vi "Scratch.vi"() -> ()   [LabVIEW 2020, in "VolatusSeq.lvlib"]
uses:
  VolatusSeq.lvlib
  Sequencing Status JSON.ctl
  Sequence Status JSON.ctl
  lv-web-crypto/lv-crypto/Crypto/Hashes/SHA-256/SHA-256.lvclass
  <vilib>/httpClient/MultipartData.ctl
  839e7588-aafe-4656-a2fc-0ebd197a9b7a.vi
  9333b484-011f-4693-912f-1257e8b2ee91.vi
  d0b18555-7aa2-4285-8466-e3de5a6bf30b.vi
  80ab21ca-ea82-40af-a504-7941cea15b69.vi
  <vilib>/JDP Science/JSONtext/Next JSON Value.vi
  <vilib>/JDP Science/JSONtext/String Subset.vi
  <vilib>/JDP Science/JSONtext/Parsing/Advance past next JSON Value (inlined COPY).vi
  <vilib>/JDP Science/JSONtext/Parsing/Advance past whitespace.vi
  <vilib>/JDP Science/JSONtext/Parsing/Advance past String.vi
  <vilib>/JDP Science/JSONtext/Parsing/Advance past Number.vi
  <vilib>/JDP Science/JSONtext/Parsing/Advance past Line Ending.vi
  <vilib>/JDP Science/JSONtext/Parsing/Parse Full Path or Item Name.vi
  <vilib>/JDP Science/JSONtext/Parsing/Advance past Array.vi
  <vilib>/JDP Science/JSONtext/Parsing/Advance past Object.vi
  <vilib>/JDP Science/JSONtext/support/Error Cluster From Code.vi
  <vilib>/JDP Science/JSONtext/Offset/Find Item Locations by Path.vi
  <vilib>/JDP Science/JSONtext/JSON text to Variant.vi
  <vilib>/JDP Science/JSONtext/LVClass Serializer/JSONtext LVClass Serializer.lvclass
  <vilib>/JDP Science/JSONtext/JSONtext.lvlib
  lv-web-crypto/lv-crypto/Crypto/Crypto.lvlib
  <vilib>/httpClient/LabVIEWHTTPClient.lvlib
  lv-vecto/Vecto/Vecto.lvlib
  lv-web-crypto/lv-json/JSON/JSON.lvlib
  ad4a9e69-8c40-4036-95cd-164e8a1331be.vi
panel:
  in  "URL Base":string="http://localhost:13083"
  out "Table":string[][](table)
  in  "Abort":bool
  in  "Unload":bool
  in  "Start":bool
  in  "Load":bool
  in  "VSEQ":string="{\n    \"Sequence\": {\n        \"Name\": \"Bottle Condition\",\n        \"Version\": \"1\",\n        \"Comment\": \"Control state machine for bottle heating/cooling.\",\n        \"Entry\": \"Start\",\n        \"Abort\": \"Stop\",\n        \"States\": {\n            \"Start\": {\n                \"Comment\": \"Reset bottle controls to off state.\",\n                \"Steps\": [\n                    {\n                        \"Time\": 0,\n                        \"Commands\": [\n                            {\"Type\": \"Transition\", \"Target\": \"Hold\"}\n                        ]\n                    }\n                ]\n            },\n            \"Hold\": {\n                \"Comment\": \"Bottle in range, controls off.\",\n                \"Steps\": [\n                    {\n                        \"Time\": 0,\n                        \"Commands\": [\n                            {\"Type\": \"Digital\", \"Channel\": \"BottleCool\", \"Value\": false},\n                            {\"Type\": \"Digital\", \"Channel\": \"BottleHeat\", \"Value\": false}\n                        ]\n                    }\n                ],\n                \"Transitions\": [\n                    {\n                        \"Type\": \"State\",\n                        \"Target\": \"Cool\",\n                        \"Logic\": \"Any\",\n                        \"Conditions\": [\n                            {\"Type\": \"HighLimit\", \"Channel\": \"BottlePSI\", \"Limit\": 850}\n                        ]\n                    },\n                    {\n                        \"Type\": \"State\",\n                        \"Target\": \"Heat\",\n                        \"Logic\": \"Any\",\n                        \"Conditions\": [\n                            {\"Type\": \"LowLimit\", \"Channel\": \"BottlePSI\", \"Limit\": 750}\n                        ]\n                    }\n                ]\n            },\n            \"Cool\": {\n                \"Comment\": \"Cooling, wait for pressure to drop.\",\n                \"Steps\": [\n                    {\n                        \"Time\": 0,\n                        \"Commands\": [\n                            {\"Type\": \"Digital\", \"Channel\": \"BottleCool\", \"Value\": true}\n                        ]\n                    }\n                ],\n                \"Transitions\": [\n                    {\n                        \"Type\": \"State\",\n                        \"Target\": \"Start\",\n                        \"Logic\": \"Any\",\n                        \"Conditions\": [\n                            {\"Type\": \"LowLimit\", \"Channel\": \"BottlePSI\", \"Limit\": 800}\n                        ]\n                    }\n                ]\n            },\n            \"Heat\": {\n                \"Comment\": \"Heating, wait for pressure to rise.\",\n                \"Steps\": [\n                    {\n                        \"Time\": 0,\n                        \"Commands\": [\n                            {\"Type\": \"Digital\", \"Channel\": \"BottleHeat\", \"Value\": true}\n                        ]\n                    }\n                ],\n                \"Transitions\": [\n                    {\n                        \"Type\": \"State\",\n                        \"Target\": \"Start\",\n                        \"Logic\": \"Any\",\n                        \"Conditions\": [\n                            {\"Type\": \"HighLimit\", \"Channel\": \"BottlePSI\", \"Limit\": 800}\n                        ]\n                    }\n                ]\n            },\n            \"Stop\": {\n                \"Comment\": \"Stopping, ensure controls off.\",\n                \"Steps\": [\n                    {\n                        \"Time\": 0,\n                        \"Commands\": [\n                            {\"Type\": \"Digital\", \"Channel\": \"BottleCool\", \"Value\": false},\n                            {\"Type\": \"Digital\", \"Channel\": \"BottleHeat\", \"Value\": false},\n                            {\"Type\": \"Stop\"}\n                        ]\n                    }\n                ]\n            }\n        }\n    }\n}"
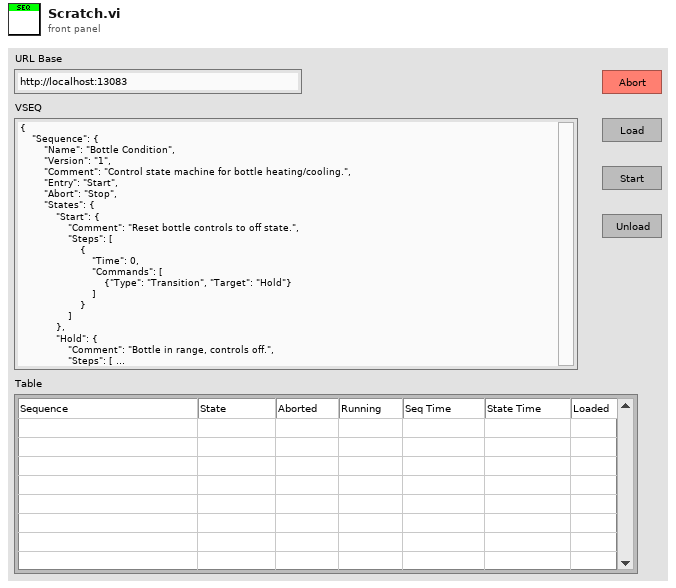
[diagram p1: front panel]
types:
  T1 = typedef "VolatusSeq.lvlib/Sequencing Status JSON.ctl" = cluster{"sequences":T2[]}
  T2 = typedef "VolatusSeq.lvlib/Sequence Status JSON.ctl" = cluster{"name":string, "state":string, "running":bool, "abort":bool, "time":cluster{"seq":i64, "state":i64, "wall":i64}, "loaded":bool, "started":i64, "crc":u32, "color_bg":string, "color_fg":string}
  T3 = typedef "LabVIEWHTTPClient.lvlib/MultipartData.ctl" = cluster{"Name":string, "Value":string, "File":path, "Filename":string, "MIME type":string}
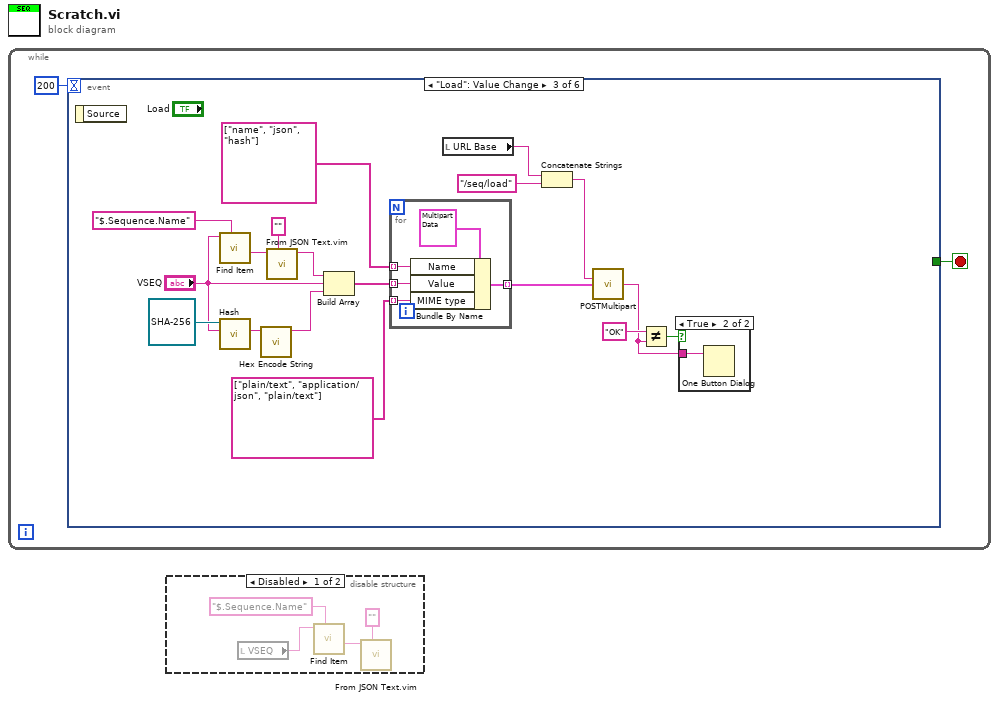
[diagram p0: block diagram]
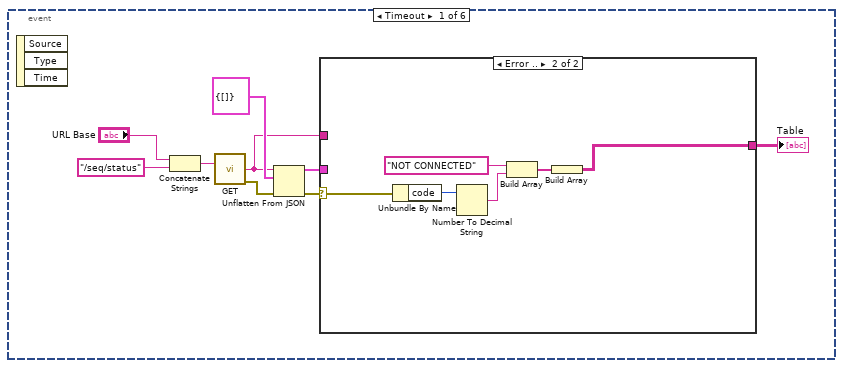
[diagram p3: hidden frame]
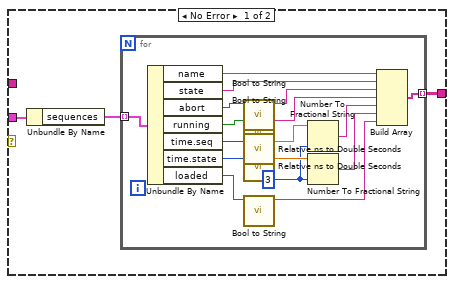
[diagram p4: hidden frame]
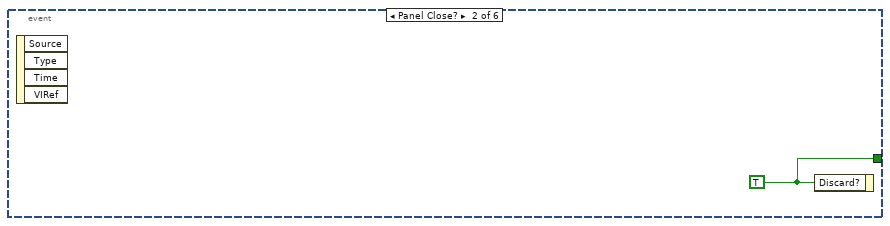
[diagram p5: hidden frame]
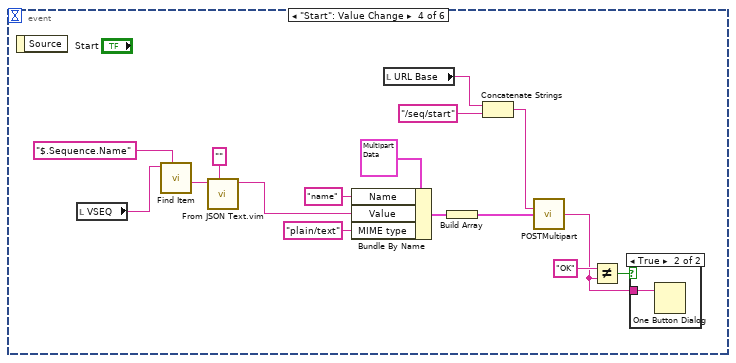
[diagram p7: hidden frame]
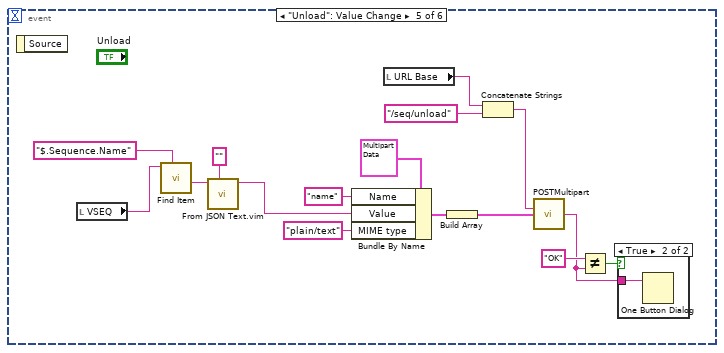
[diagram p9: hidden frame]
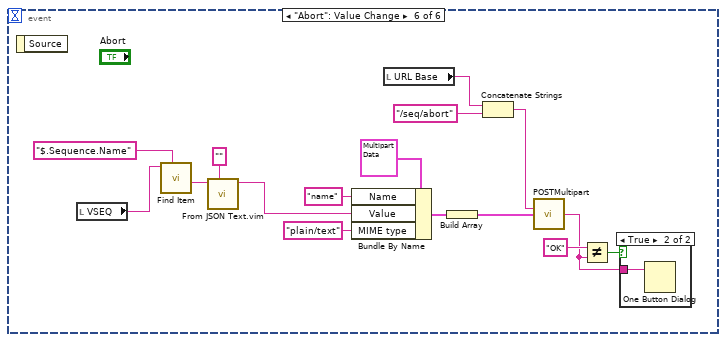
[diagram p11: hidden frame]
diagram:
  n1 = while {
    stop <- w1 stop-if-true
    n2 = event shown="[2] \"Load\": Value Change" {
      selector: _ -> [_ _ _ _ _ _]
      dyn-events: _ -> [_ _ _ _ _ _]
      timeout: 200 -> [_ _ _ _ _ _]
      tunnel: [_ w38 _ _ _ _] -> w1
      event Timeout {
        n3 = event-data() -> ()  [unwired: 1 in, 3 out]
        n4 = Concatenate Strings("URL Base", "/seq/status" ("string")) -> (w9:string)
        n5 = call <vilib>:"GET.vi"("url"=w9) -> ("body"=w3:string, "error out"=w8:errorcluster)  [unwired: 11 in, 2 out]
        n6 = Unflatten From JSON(JSON string=w3, type and defaults=T1 {"sequences"=[]} ("Sequencing Status JSON"), error in (no error)=w8) -> (value=w6:T1, error out=w4:errorcluster)  [unwired: 4 in]
        n7 = case shown="Error .." w4 {
          selector: w4 -> [_ w37]
          tunnel: w6 -> [w14 _]
          tunnel: [w12 w32] -> w5
          tunnel: w3 -> [_ _]
          frame No Error {
            n8 = Unbundle By Name(w14) -> ("sequences"=w13:T2[])
            n9 = for {
              tunnel: w13 -> [w31] mode=indexing
              tunnel: [w17] -> w12 mode=indexing
              w25 = i16 3 ("precision (6)")
              n10 = Unbundle By Name(w31) -> ("name"=w23:string, "state"=w22:string, "abort"=w28:bool, "running"=w27:bool, "time.seq"=w30:i64, "time.state"=w29:i64, "loaded"=w16:bool)
              n11 = call "Bool to String.vi"("Boolean"=w28) -> ("Value"=w21:string)  [unwired: 10 in]
              n12 = call "Bool to String.vi"("Boolean"=w27) -> ("Value"=w20:string)  [unwired: 10 in]
              n13 = call "Relative ns to Double Seconds.vi"("relative ns"=w30) -> ("Double s"=w24:dbl)  [unwired: 6 in]
              n14 = call "Relative ns to Double Seconds.vi"("relative ns"=w29) -> ("Double s"=w26:dbl)  [unwired: 6 in]
              n15 = call "Bool to String.vi"("Boolean"=w16) -> ("Value"=w15:string)  [unwired: 10 in]
              n16 = Number To Fractional String(number=w24, precision (6)=w25) -> (F-format string=w19:string)  [unwired: 2 in]
              n17 = Number To Fractional String(number=w26, precision (6)=w25) -> (F-format string=w18:string)  [unwired: 2 in]
              n18 = Build Array(w23, w22, w21, w20, w19, w18, w15) -> (w17:string[])
            }
          }
          frame Error {
            n19 = Unbundle By Name(w37) -> ("code"=w36:i32)
            n20 = Number To Decimal String(number=w36) -> (decimal integer string=w34:string)  [unwired: 1 in]
            n21 = Build Array("NOT CONNECTED", w34) -> (w33:string[])
            n22 = Build Array(w33) -> (w32:string[][])
          }
        }
        "Table" <- w5
      }
      event Panel Close? {
        w38 = TRUE ("Discard?")
        n23 = event-data() -> ()  [unwired: 1 in, 4 out]
        n24 = event-data("Discard?"=w38) -> ()  [unwired: 1 in, 1 out]
      }
      event "Load": Value Change {
        n25 = event-data() -> ()  [unwired: 1 in, 1 out]
        n26 = call <vilib>:"Find Item.vi"("$Path or Item Name"="$.Sequence.Name", "JSON"="VSEQ") -> ("<JSON>"=w56:string)  [unwired: 6 in, 3 out]
        n27 = call-dynamic "Hash.vi"("Message"="VSEQ", "SHA-256 in"=refnum<class "SHA-256.lvclass"> refnum) -> ("Hash"=w55:string)  [unwired: 7 in, 2 out]
        n28 = call "Hex Encode String.vi"("String"=w55) -> ("Hex Encoded String"=w49:string)  [unwired: 10 in]
        n29 = call "From JSON Text.vim"("Data Type and Default Value"="", "JSON"=w56) -> ("Data out"=w51:string)  [unwired: 8 in, 1 out]
        n30 = Build Array(w51, "VSEQ", w49) -> (w48:string[])
        n31 = for {
          tunnel: w48 -> [w61] mode=indexing
          tunnel: string[] ["name", "json", "hash"] -> [w60] mode=indexing
          tunnel: string[] ["plain/text", "application/json", "plain/text"] -> [w59] mode=indexing
          tunnel: [w58] -> w45 mode=indexing
          n32 = Bundle By Name(cluster=T3 {"Name"="", "Value"="", "File"=path "", "Filename"="", "MIME type"="application/octet-stream"} ("Element"), "Name"=w60, "Value"=w61, "MIME type"=w59) -> (w58:T3)
        }
        n33 = local read "URL Base"() -> (w44:string)
        n34 = Concatenate Strings(w44, "/seq/load" ("string")) -> (w42:string)
        n35 = call <vilib>:"POSTMultipart.vi"("url"=w42, "data"=w45) -> ("body"=w39:string)  [unwired: 10 in, 3 out]
        n36 = Not Equal?(x="OK", y=w39) -> (x != y?=w40:bool)
        n37 = case shown="True" w40 {
          tunnel: w39 -> [_ w57]
          frame False {
          }
          frame True {
            n38 = One Button Dialog(message=w57) -> ()  [unwired: 1 in, 1 out]
          }
        }
      }
      event "Start": Value Change {
        n39 = event-data() -> ()  [unwired: 1 in, 1 out]
        n40 = local read "VSEQ"() -> (w72:string)
        n41 = call <vilib>:"Find Item.vi"("$Path or Item Name"="$.Sequence.Name", "JSON"=w72) -> ("<JSON>"=w78:string)  [unwired: 6 in, 3 out]
        n42 = call "From JSON Text.vim"("Data Type and Default Value"="", "JSON"=w78) -> ("Data out"=w68:string)  [unwired: 8 in, 1 out]
        n43 = Bundle By Name(cluster=T3 {"Name"="", "Value"="", "File"=path "", "Filename"="", "MIME type"="application/octet-stream"} ("Element"), "Name"="name", "Value"=w68, "MIME type"="plain/text") -> (w67:T3)
        n44 = local read "URL Base"() -> (w75:string)
        n45 = Build Array(w67) -> (w66:T3[])
        n46 = Concatenate Strings(w75, "/seq/start" ("string")) -> (w73:string)
        n47 = call <vilib>:"POSTMultipart.vi"("url"=w73, "data"=w66) -> ("body"=w63:string)  [unwired: 10 in, 3 out]
        n48 = Not Equal?(x="OK", y=w63) -> (x != y?=w64:bool)
        n49 = case shown="True" w64 {
          tunnel: w63 -> [_ w79]
          frame False {
          }
          frame True {
            n50 = One Button Dialog(message=w79) -> ()  [unwired: 1 in, 1 out]
          }
        }
      }
      event "Unload": Value Change {
        n51 = event-data() -> ()  [unwired: 1 in, 1 out]
        n52 = local read "VSEQ"() -> (w89:string)
        n53 = call <vilib>:"Find Item.vi"("$Path or Item Name"="$.Sequence.Name", "JSON"=w89) -> ("<JSON>"=w95:string)  [unwired: 6 in, 3 out]
        n54 = call "From JSON Text.vim"("Data Type and Default Value"="", "JSON"=w95) -> ("Data out"=w85:string)  [unwired: 8 in, 1 out]
        n55 = Bundle By Name(cluster=T3 {"Name"="", "Value"="", "File"=path "", "Filename"="", "MIME type"="application/octet-stream"} ("Element"), "Name"="name", "Value"=w85, "MIME type"="plain/text") -> (w84:T3)
        n56 = local read "URL Base"() -> (w92:string)
        n57 = Build Array(w84) -> (w83:T3[])
        n58 = Concatenate Strings(w92, "/seq/unload" ("string")) -> (w90:string)
        n59 = call <vilib>:"POSTMultipart.vi"("url"=w90, "data"=w83) -> ("body"=w80:string)  [unwired: 10 in, 3 out]
        n60 = Not Equal?(x="OK", y=w80) -> (x != y?=w81:bool)
        n61 = case shown="True" w81 {
          tunnel: w80 -> [_ w96]
          frame False {
          }
          frame True {
            n62 = One Button Dialog(message=w96) -> ()  [unwired: 1 in, 1 out]
          }
        }
      }
      event "Abort": Value Change {
        n63 = event-data() -> ()  [unwired: 1 in, 1 out]
        n64 = local read "VSEQ"() -> (w106:string)
        n65 = call <vilib>:"Find Item.vi"("$Path or Item Name"="$.Sequence.Name", "JSON"=w106) -> ("<JSON>"=w112:string)  [unwired: 6 in, 3 out]
        n66 = call "From JSON Text.vim"("Data Type and Default Value"="", "JSON"=w112) -> ("Data out"=w102:string)  [unwired: 8 in, 1 out]
        n67 = Bundle By Name(cluster=T3 {"Name"="", "Value"="", "File"=path "", "Filename"="", "MIME type"="application/octet-stream"} ("Element"), "Name"="name", "Value"=w102, "MIME type"="plain/text") -> (w101:T3)
        n68 = local read "URL Base"() -> (w109:string)
        n69 = Build Array(w101) -> (w100:T3[])
        n70 = Concatenate Strings(w109, "/seq/abort" ("string")) -> (w107:string)
        n71 = call <vilib>:"POSTMultipart.vi"("url"=w107, "data"=w100) -> ("body"=w97:string)  [unwired: 10 in, 3 out]
        n72 = Not Equal?(x="OK", y=w97) -> (x != y?=w98:bool)
        n73 = case shown="True" w98 {
          tunnel: w97 -> [_ w113]
          frame False {
          }
          frame True {
            n74 = One Button Dialog(message=w113) -> ()  [unwired: 1 in, 1 out]
          }
        }
      }
    }
  }
  n75 = disable-structure shown="Disabled" {
    frame Disabled {
      n76 = local read "VSEQ"() -> (w114:string)
      n77 = call <vilib>:"Find Item.vi"("$Path or Item Name"="$.Sequence.Name", "JSON"=w114) -> ("<JSON>"=w115:string)  [unwired: 6 in, 3 out]
      n78 = call "From JSON Text.vim"("Data Type and Default Value"="", "JSON"=w115) -> ()  [unwired: 8 in, 2 out]
    }
    frame Enabled {
    }
  }
